vi "Initialize MeasurementLink Session.vi"(7 "remote connection options":T2, 8 "error in":errorcluster, 9 "initialize and close session behavior":T1, 10 "session initialization parameters":T3, 11 "session factory in":refnum<class "Session Factory.lvclass">) -> (0 "error out":errorcluster, 2 "session out":variant, 3 "session factory out":refnum<class "Session Factory.lvclass">)   [LabVIEW 2021, in "NI Session Management niDigital.lvlib" / "Session Factory.lvclass"]
uses:
  Session Factory.lvclass
  Instrument/ISession Factory/Session Initialization Parameters.ctl
  Instrument/ISession Factory/Remote Connection Options.ctl
  Instrument/ISession Factory/Initialize and Close Session Behavior.ctl
  Session Factory.lvclass/Session Factory.ctl
  Instrument/ISession Factory/ISession Factory.lvclass
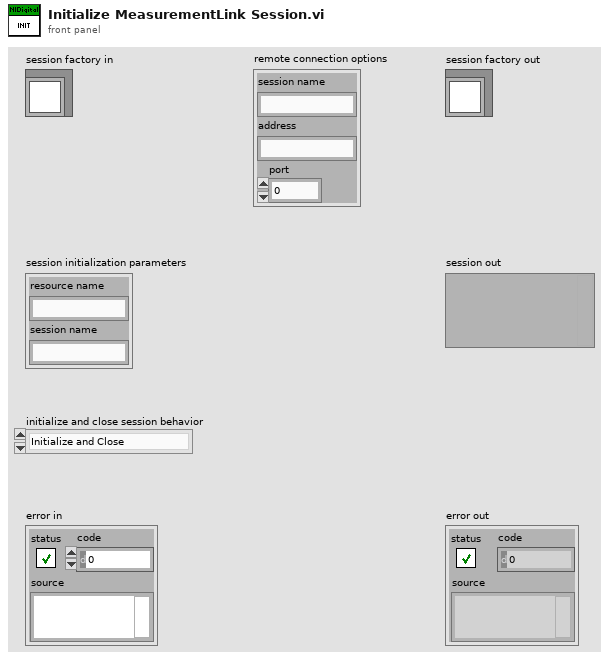
[diagram p1: front panel]
types:
  T1 = typedef "NI Session Management Instrument.lvlib/ISession Factory.lvclass/Initialize and Close Session Behavior.ctl" = enum16{"Initialize and Close", "Attach and Detach", "Initialize and Detach", "Attach and Close"}
  T2 = typedef "NI Session Management Instrument.lvlib/ISession Factory.lvclass/Remote Connection Options.ctl" = cluster{"session name":string, "address":string, "port":u32}
  T3 = typedef "NI Session Management Instrument.lvlib/ISession Factory.lvclass/Session Initialization Parameters.ctl" = cluster{"resource name":string, "session name":string}
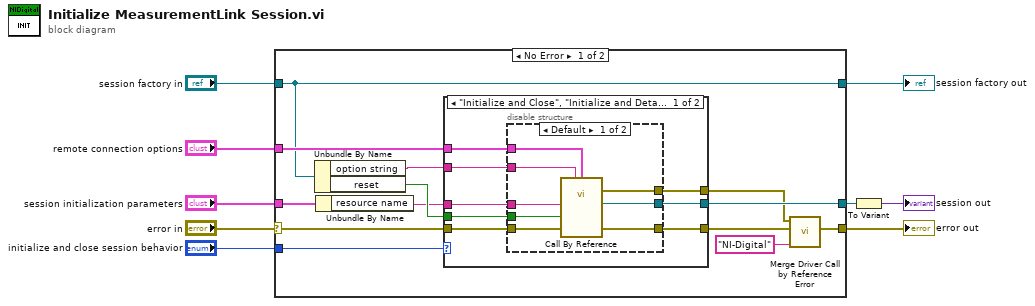
[diagram p0: block diagram]
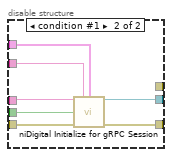
[diagram p2: hidden frame]
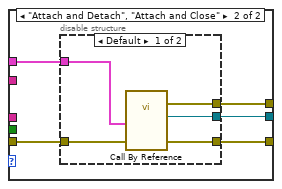
[diagram p3: hidden frame]
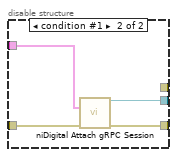
[diagram p4: hidden frame]
diagram:
  n1 = case shown="No Error" "error in" {
    selector: "error in" -> [w19 w60]
    tunnel: [w12 w60] -> w8
    tunnel: "session factory in" -> [w17 w61]
    tunnel: [w17 w61] -> w6
    tunnel: "initialize and close session behavior" -> [w22 _]
    tunnel: "remote connection options" -> [w21 _]
    tunnel: "session initialization parameters" -> [w18 _]
    tunnel: [w20 _] -> w2
    frame No Error {
      n2 = Unbundle By Name(w17) -> ("option string"=w16:string, "reset"=w15:bool)
      n3 = Unbundle By Name(w18) -> ("resource name"=w14:string)
      n4 = case shown="\"Initialize and Close\", \"Initialize and Detach\"" w22 {
        tunnel: w21 -> [w29 w50]
        tunnel: [w28 w49] -> w20
        tunnel: w19 -> [w30 w48]
        tunnel: [w27 w47] -> w13
        tunnel: w14 -> [w26 _]
        tunnel: w16 -> [w25 _]
        tunnel: w15 -> [w24 _]
        tunnel: [w23 w46] -> w11
        frame "Initialize and Close", "Initialize and Detach" {
          n5 = disable-structure shown="Default" {
            disable-tunnel: w30 -> [w38 w45]
            disable-tunnel: w29 -> [w37 w40]
            disable-tunnel: [w36 w43] -> w28
            disable-tunnel: [w35 w44] -> w27
            disable-tunnel: w26 -> [w34 w42]
            disable-tunnel: w25 -> [w33 w39]
            disable-tunnel: w24 -> [w32 w41]
            disable-tunnel: [w31 _] -> w23
            frame condition #0 (active) {
              n6 = call-by-ref "?"("resource name"=w34, "option string"=w33, "gRPC options"=w37, "reset (F)"=w32, "error in"=w38) -> (error out=w31:errorcluster, "instrument handle"=w36:refnum<k15>, 15:"error out"=w35:errorcluster)  [unwired: 11 in, 1 out]
            }
            frame condition #1 {
              n7 = call <instrlib>:"niDigital Initialize for gRPC Session.vi"("resource name"=w42, "option string"=w39, "gRPC options"=w40, "reset (F)"=w41, "error in"=w45) -> ("instrument handle"=w43:refnum<k15>, "error out"=w44:errorcluster)  [unwired: 9 in]
            }
          }
        }
        frame "Attach and Detach", "Attach and Close" {
          n8 = disable-structure shown="Default" {
            disable-tunnel: w50 -> [w55 w56]
            disable-tunnel: [w54 w57] -> w49
            disable-tunnel: w48 -> [w53 w59]
            disable-tunnel: [w52 w58] -> w47
            disable-tunnel: [w51 _] -> w46
            frame condition #0 (active) {
              n9 = call-by-ref "?"("gRPC options"=w55, "error in"=w53) -> (error out=w51:errorcluster, "instrument handle out"=w54:refnum<k15>, 15:"error out"=w52:errorcluster)  [unwired: 14 in, 1 out]
            }
            frame condition #1 {
              n10 = call <instrlib>:"niDigital Attach gRPC Session.vi"("gRPC options"=w56, "error in"=w59) -> ("instrument handle out"=w57:refnum<k15>, "error out"=w58:errorcluster)  [unwired: 12 in]
            }
          }
        }
      }
      n11 = call "Merge Driver Call by Reference Error.vi"("driver name"="NI-Digital", "called vi error"=w13, "call by ref error"=w11) -> ("error out"=w12:errorcluster)  [unwired: 8 in]
    }
    frame Error {
    }
  }
  "error out" <- w8
  "session factory out" <- w6
  n12 = To Variant(anything=w2) -> (Variant=→"session out":variant)
